vi "Wire 2 terminal function.vi"(5 "Sink":refnum<vi>, 8 "error in (no error)":errorcluster, 10 "Source":refnum<vi>, 11 "2 Terminal Function In":refnum<vi>) -> (0 "error out":errorcluster, 2 "Output Terminal":refnum<vi>, 3 "2 Terminal Function Out":refnum<vi>)   [LabVIEW 2012, in "Scripting Tools.lvlib"]
doc: "Wires a one input, one output function with the source and sink terminals and returns a reference to the output terminal"
uses:
  Scripting Tools.lvlib
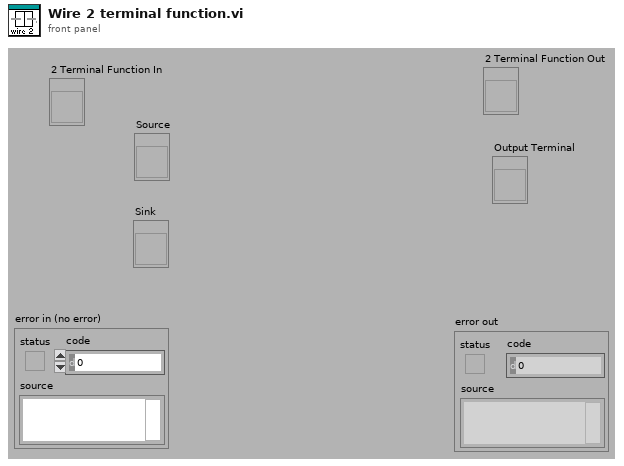
[diagram p1: front panel]
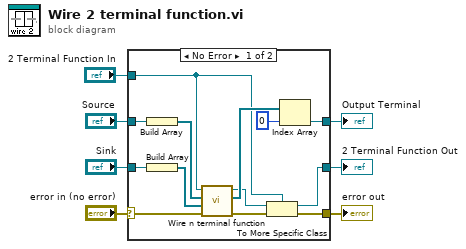
[diagram p0: block diagram]
diagram:
  n1 = case shown="No Error" "error in (no error)" {
    selector: "error in (no error)" -> [w10 w22]
    tunnel: [w8 w22] -> w7
    tunnel: "Sink" -> [w20 _]
    tunnel: "Source" -> [w18 _]
    tunnel: [w14 _] -> w4
    tunnel: [w12 w21] -> w3
    tunnel: "2 Terminal Function In" -> [w11 w21]
    frame No Error {
      n2 = Build Array(w18) -> (w17:refnum<vi>[])
      n3 = Build Array(w20) -> (w19:refnum<vi>[])
      n4 = call "Wire n terminal function.vi"("error in (no error)"=w10, "Sink Terminals"=w19, "Source Terminals"=w17, "Node In"=w11) -> ("error out"=w9:errorcluster, "Function Output Terminals"=w16:refnum<vi>[], "Node Out"=w13:refnum<vi>)  [unwired: 5 out]
      n5 = To More Specific Class(target class=w11, reference=w13, error in=w9) -> (specific class reference=w12:refnum<vi>, error out=w8:errorcluster)
      n6 = Index Array(array=w16, index=0) -> (element=w14:refnum<vi>)
    }
    frame Error {
    }
  }
  "2 Terminal Function Out" <- w3
  "error out" <- w7
  "Output Terminal" <- w4
